vi "ParamsMeasure.vi"(3 "InputData":u8[](array[numeric])=[154, 153, 153, 63, 6, 0, 1, 1, 0, 0, 72, 68, 6, 255, 1, 1, 205, 204, 140, 63, 6, 0, 1, 1, 0, 0, 97, 68, 6, 255, 1, 1, 0, 0, 72, 68, 6, 255, 1, 1, 0, 0, 200, 67, 6, 255, 1, 1, 0, 0, 198, 67, 6, 255, 1, 1, 0, 0, 128, 63, 6, 0, 1, 1, 0, 0, 0, 0, 255, 0, 0, 0, 227, 231, 129, 63, 6, 0, 1, 1, 0, 0, 0, 0, 255, 0, 0, 0, 0, 0, 0, 0, 255, 0, 0, 0, 0, 0, 0, 0, 255, 0, 0, 0, 255, 255, 127, 127, 10, 0, 0, 1, 255, 255, 127, 127, 10, 0, 0, 1, 255, 255, 127, 127, 1, 254, 0, 1, 255, 255, 127, 127, 0, 2, 0, 1, 255, 255, 127, 127, 1, 254, 0, 1, 255, 255, 127, 127, 1, 254, 0, 1, 255, 255, 127, 127, 1, 254, 0, 1, 255, 255, 127, 127, 1, 254, 0, 1, 255, 255, 127, 127, 10, 0, 0, 1, 255, 255, 127, 127, 10, 0, 0, 1, 0, 0, 0, 0, 255, 0, 0, 0, 0, 0, 0, 0, 255, 0, 0, 0, 0, 0, 0, 0, 255, 0, 0, 0, 0, 0, 0, 0, 255, 0, 0, 0, 0, 0, 0, 0, 255, 0, 0, 0, 0, 0, 0, 0, 255, 0, 0, 0, 0, 0, 0, 0, 255, 0, 0, 0, 0, 0, 0, 0, 255, 0, 0, 0, 0, 0, 0, 0, 255, 0, 0, 0, 0, 0, 0, 0, 255, 0, 0, 0, 0, 0, 0, 0, 255, 0, 0, 0, 0, 0, 0, 0, 255, 0, 0, 0, 0, 0, 0, 0, 255, 0, 0, 0, 0, 0, 0, 0, 255, 0, 0, 0, 0, 0, 0, 0, 255, 0, 0, 0, 0, 0, 0, 0, 255, 0, 0, 0, 0, 0, 0, 0, 255, 0, 0, 0, 0, 0, 0, 0, 255, 0, 0, 0, 0, 0, 0, 0, 255, 0, 0, 0, 0, 0, 0, 0, 255, 0, 0, 0, 0, 0, 0, 0, 255, 0, 0, 0, 0, 0, 0, 0, 255, 0, 0, 0, 0, 0, 0, 0, 255, 0, 0, 0, 0, 0, 0, 0, 255, 0, 0, 0, 0, 0, 0, 0, 255, 0, 0, 0, 0, 0, 0, 0, 255, 0, 0, 0, 0, 0, 0, 0, 255, 0, 0, 0] format="%02x", 6 "UCI_DllPath":path=path "E:/JL-Project/LabView-Project/ASCII/uci.dll") -> (0 "OuputData":sgl[](array[numeric]), 2 "OutputString":string)   [LabVIEW 2015]
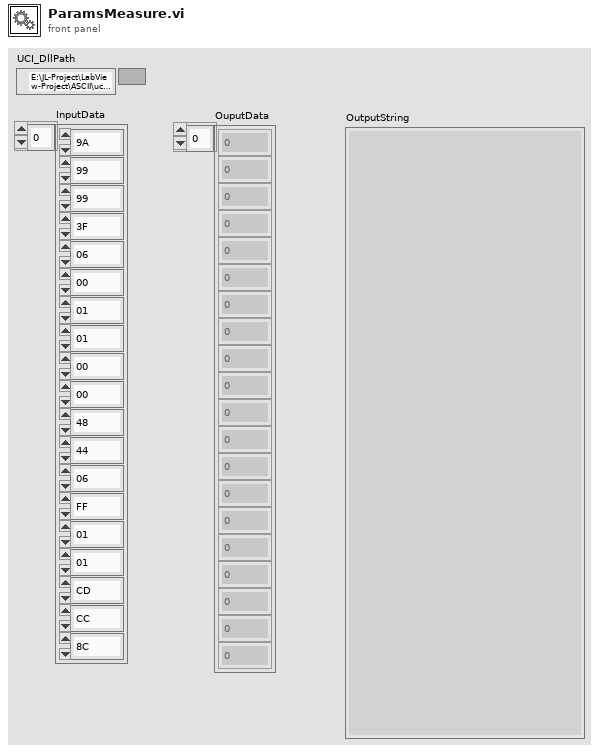
[diagram p1: front panel]
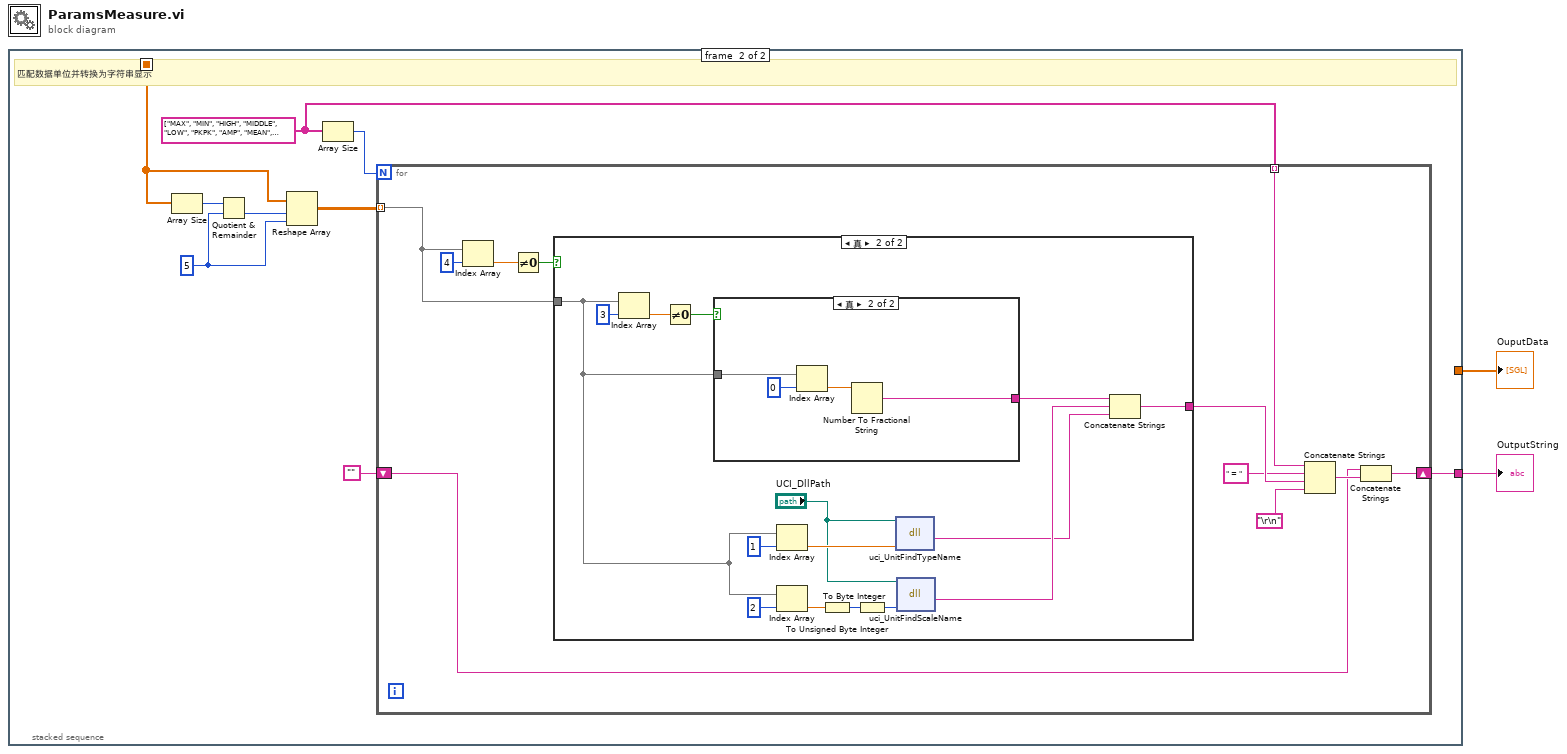
[diagram p0: block diagram]
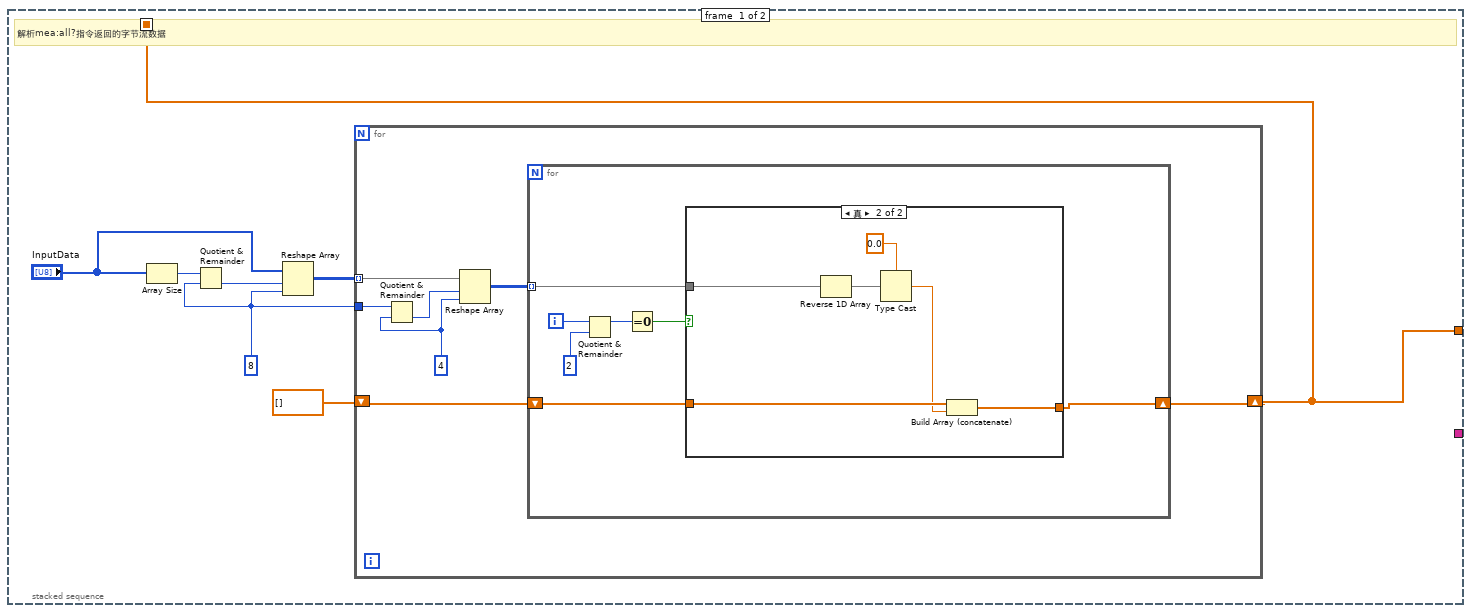
[diagram p2: hidden frame]
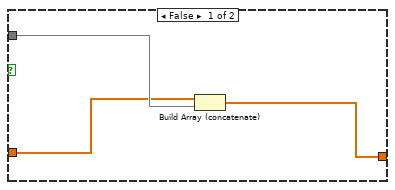
[diagram p3: hidden frame]
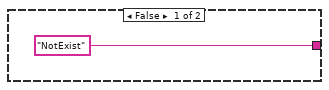
[diagram p4: hidden frame]
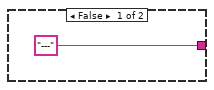
[diagram p5: hidden frame]
diagram:
  n1 = stacked-sequence {
    seq-local: [w3 _] -> [_ w38]
    tunnel: [_ w34] -> w2
    tunnel: [w3 _] -> w1
    frame #0 {
      w7 = 8 ("维数大小")
      # "解析mea:all?指令返回的字节流数据"
      n2 = Array Size(array="InputData") -> (size(s)=w9:i32)
      n3 = Quotient & Remainder(x=w9, y=w7) -> (floor(x/y)=w5:i32)  [unwired: 1 out]
      n4 = Reshape Array("InputData", w5, w7) -> (w8:u8[][])
      n5 = for {
        tunnel: w8 -> [w16] mode=indexing
        tunnel: w7 -> [w15]
        shift-right: [w10] -> w3
        shift-left: sgl[] [] -> [w11]
        w14 = 4 ("维数大小")
        n6 = Quotient & Remainder(x=w15, y=w14) -> (floor(x/y)=w13:i32)  [unwired: 1 out]
        n7 = Reshape Array(w16, w13, w14) -> (w12:u8[][])
        n8 = for {
          tunnel: w12 -> [w20] mode=indexing
          shift-right: [w17] -> w10
          shift-left: w11 -> [w18]
          i -> [w23]
          n9 = Quotient & Remainder(x=w23, y=2) -> (x-y*floor(x/y)=w19:i32)  [unwired: 1 out]
          n10 = Equal To 0?(x=w19) -> (x = 0?=w21:bool)
          n11 = case shown="真" w21 {
            tunnel: w20 -> [w26 w32]
            tunnel: w18 -> [w25 w29]
            tunnel: [w24 w27] -> w17
            frame False {
              n12 = Build Array (concatenate)(w25, w26) -> (w24:sgl[])
            }
            frame True {
              n13 = Reverse 1D Array(array=w32) -> (reversed array=w30:u8[])
              n14 = Type Cast(type=sgl 0.0 ("类型"), x=w30) -> (*(type *) &x=w28:sgl)
              n15 = Build Array (concatenate)(w29, w28) -> (w27:sgl[])
            }
          }
        }
      }
    }
    frame #1 {
      w35 = string[] ["MAX", "MIN", "HIGH", "MIDDLE", "LOW", "PKPK", "AMP", "MEAN", "CYCMEAN", "RMS", "CYCRMS", "AREA", "CYCAREA", "OVERSHOOT", "PRESHOOT", "PERIOD", "FREQ", "RISE_TIME", "FALL_TIME", "PWIDTH", "NWIDTH", "PDUTY", "NDUTY", "RISEDELAY", "FALLDELAY", "PHASE", "FRR", "FRF", "FFR", "FFF", "LRF", "LRR", "LFR", "LFF", "BURST_WIDTH"]
      w39 = 5 ("索引")
      # "匹配数据单位并转换为字符串显示"
      n16 = Array Size(array=w38) -> (size(s)=w41:i32)
      n17 = Quotient & Remainder(x=w41, y=w39) -> (floor(x/y)=w40:i32)  [unwired: 1 out]
      n18 = Reshape Array(w38, w40, w39) -> (w37:sgl[][])
      n19 = Array Size(array=w35) -> (size(s)=w36:i32)
      n20 = for {
        N: w36 -> [_]
        tunnel: w37 -> [w49] mode=indexing
        tunnel: w35 -> [w45] mode=indexing
        shift-right: [w43] -> w34
        shift-left: "" -> [w42]
        n21 = Index Array(array=w49, index=4 ("索引")) -> (element=w51:sgl)
        n22 = Not Equal To 0?(x=w51) -> (x != 0?=w50:bool)
        n23 = case shown="真" w50 {
          tunnel: w49 -> [_ w56]
          tunnel: ["NotExist" w54] -> w48
          frame False {
          }
          frame True {
            n24 = Index Array(array=w56, index=3 ("索引")) -> (element=w67:sgl)
            n25 = Not Equal To 0?(x=w67) -> (x != 0?=w66:bool)
            n26 = case shown="真" w66 {
              tunnel: w56 -> [_ w71]
              tunnel: ["---" w70] -> w55
              frame False {
              }
              frame True {
                n27 = Index Array(array=w71, index=0 ("索引")) -> (element=w72:sgl)
                n28 = Number To Fractional String(number=w72) -> (F-format string=w70:string)  [unwired: 3 in]
              }
            }
            n29 = Index Array(array=w56, index=1 ("索引")) -> (element=w63:sgl)
            n30 = Index Array(array=w56, index=2 ("索引")) -> (element=w59:sgl)
            n31 = To Unsigned Byte Integer(number=w59) -> (unsigned 8bit integer=w58:u8)
            n32 = To Byte Integer(number=w58) -> (8bit integer=w57:i8)
            n33 = dll-call lib="E:/JL-Project/LabView-Project/ASCII/uci.dll" fn="uci_UnitFindTypeName"(path in="UCI_DllPath", "_code"=w63) -> ("返回类型"=w60:string)  [unwired: 3 in, 2 out]
            n34 = dll-call lib="E:/JL-Project/LabView-Project/ASCII/uci.dll" fn="uci_UnitFindScaleName"(path in="UCI_DllPath", "_code"=w57) -> ("返回类型"=w61:string)  [unwired: 3 in, 2 out]
            n35 = Concatenate Strings(w55, w61, w60) -> (w54:string)
          }
        }
        n36 = Concatenate Strings(w45, " = " ("字符串"), w48, "\r\n") -> (w44:string)
        n37 = Concatenate Strings(w42, w44) -> (w43:string)
      }
    }
  }
  "OutputString" <- w2
  "OuputData" <- w1
